vi "ModbusWirteHD220.vi"(8 "error in (no error)":errorcluster caption="에러 입력(에러 없음)", 11 "Modbus master out 2":refnum<class "Modbus Master.lvclass">) -> (0 "error out":errorcluster caption="에러 출력", 3 "Modbus master out":refnum<class "Modbus Master.lvclass">)   [LabVIEW 2019]
uses:
  <vilib>/NI/Modbus Library/API/Master/Modbus Master.lvclass
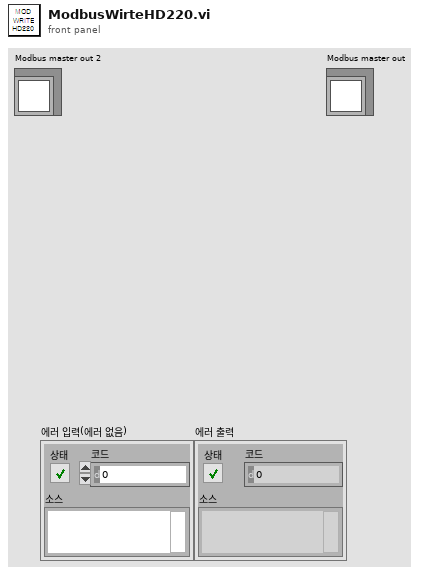
[diagram p1: front panel]
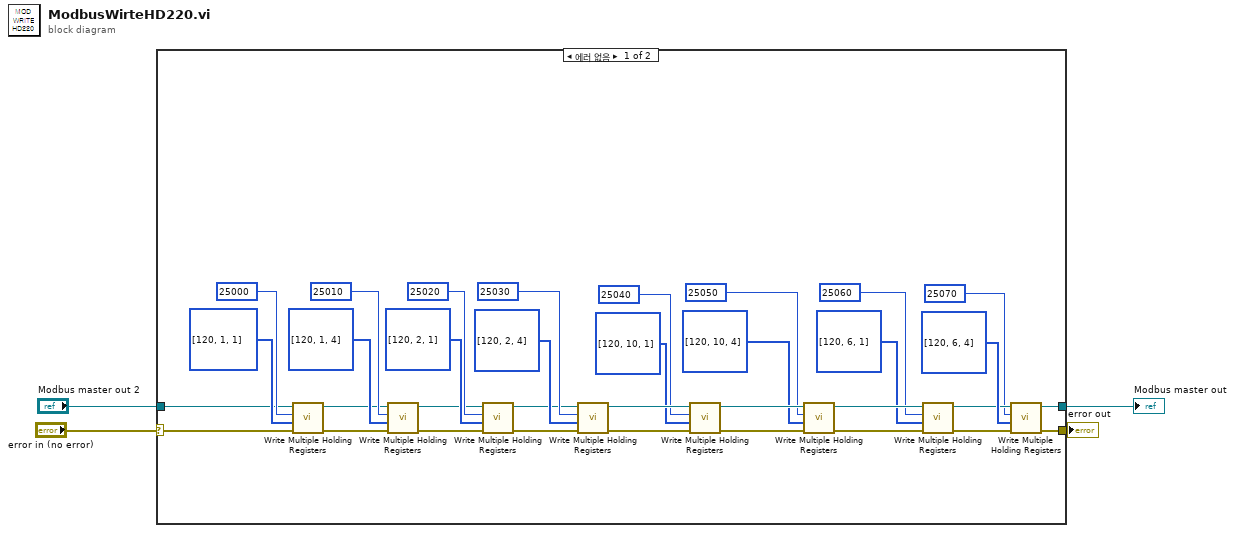
[diagram p0: block diagram]
diagram:
  n1 = case shown="에러 없음" "error in (no error)" {
    selector: "error in (no error)" -> [w15 w38]
    tunnel: [w7 w39] -> w2
    tunnel: "Modbus master out 2" -> [w14 w39]
    tunnel: [w4 w38] -> _
    frame No Error {
      n2 = call-dynamic "Write Multiple Holding Registers.vi"("error in"=w15, "registers to write"=u16[] [120, 1, 1], "starting address"=u16 25000, "Modbus master in"=w14) -> ("error out"=w37:errorcluster, "Modbus master out"=w24:refnum<class "Modbus Master.lvclass">)  [unwired: 6 in]
      n3 = call-dynamic "Write Multiple Holding Registers.vi"("error in"=w37, "registers to write"=u16[] [120, 1, 4], "starting address"=u16 25010, "Modbus master in"=w24) -> ("error out"=w36:errorcluster, "Modbus master out"=w25:refnum<class "Modbus Master.lvclass">)  [unwired: 6 in]
      n4 = call-dynamic "Write Multiple Holding Registers.vi"("error in"=w36, "registers to write"=u16[] [120, 2, 1], "starting address"=u16 25020, "Modbus master in"=w25) -> ("error out"=w35:errorcluster, "Modbus master out"=w26:refnum<class "Modbus Master.lvclass">)  [unwired: 6 in]
      n5 = call-dynamic "Write Multiple Holding Registers.vi"("error in"=w35, "registers to write"=u16[] [120, 2, 4], "starting address"=u16 25030, "Modbus master in"=w26) -> ("error out"=w16:errorcluster, "Modbus master out"=w23:refnum<class "Modbus Master.lvclass">)  [unwired: 6 in]
      n6 = call-dynamic "Write Multiple Holding Registers.vi"("error in"=w16, "registers to write"=u16[] [120, 10, 1], "starting address"=u16 25040, "Modbus master in"=w23) -> ("error out"=w17:errorcluster, "Modbus master out"=w22:refnum<class "Modbus Master.lvclass">)  [unwired: 6 in]
      n7 = call-dynamic "Write Multiple Holding Registers.vi"("error in"=w17, "registers to write"=u16[] [120, 10, 4], "starting address"=u16 25050, "Modbus master in"=w22) -> ("error out"=w12:errorcluster, "Modbus master out"=w13:refnum<class "Modbus Master.lvclass">)  [unwired: 6 in]
      n8 = call-dynamic "Write Multiple Holding Registers.vi"("error in"=w12, "registers to write"=u16[] [120, 6, 1], "starting address"=u16 25060, "Modbus master in"=w13) -> ("error out"=w11:errorcluster, "Modbus master out"=w6:refnum<class "Modbus Master.lvclass">)  [unwired: 6 in]
      n9 = call-dynamic "Write Multiple Holding Registers.vi"("error in"=w11, "registers to write"=u16[] [120, 6, 4], "starting address"=u16 25070, "Modbus master in"=w6) -> ("error out"=w4:errorcluster, "Modbus master out"=w7:refnum<class "Modbus Master.lvclass">)  [unwired: 6 in]
    }
    frame Error {
    }
  }
  "Modbus master out" <- w2
